vi "TimeSyncServ_Exec.vi"(8 "error in (no error)":errorcluster) -> ()   [LabVIEW 2019, in "PhotonVisionLib.lvlib"]
doc: "Execute a PhotonVision Time Sync Server. It listens for UDP requests from PhotonVision devices and responds with the current FPGA time.\n\nThis VI contains a loop. Do not place this in another loop.\n\nPlace this all by itself in Periodic Tasks.\n\n\nInputs:\n -- Error In -- Optional error input cluster.\n\nOutputs:\n -- <None>"
uses:
  PhotonVisionLib.lvlib
  <vilib>/Rock Robotics/WPI/ThirdParty/JAS_Junk/TrajLib/VI/Util_GetTime_U32.vi
  PhotonVision_Globals.vi
  <vilib>/Rock Robotics/WPI/ThirdParty/JAS_Junk/TrajLib/VI/Util_GetTime_U64.vi
  <vilib>/Rock Robotics/WPI/ThirdParty/JAS_Junk/TrajLib/Trajectory_Library.lvlib
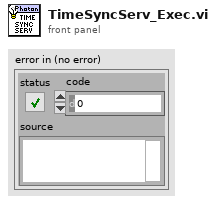
[diagram p1: front panel]
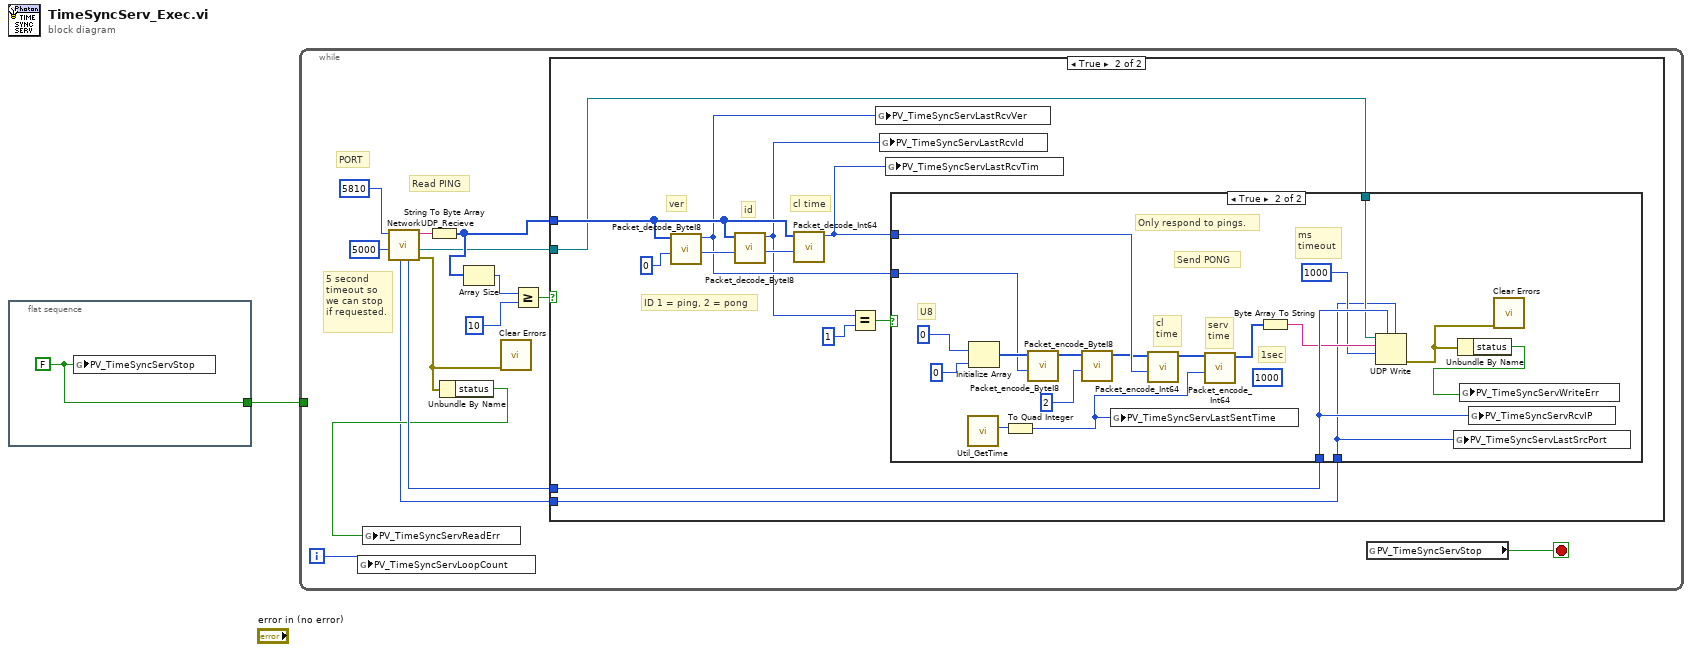
[diagram p0: block diagram]
diagram:
  n1 = flat-sequence {
    tunnel: [w2] -> w1
    frame #0 {
      w2 = FALSE ("PV_TimeSyncStopServ")
      n2 = global write "PhotonVision_Globals.vi" "PV_TimeSyncServStop"(w2) -> ()
    }
  }
  n3 = while {
    tunnel: w1 -> [_]
    i -> [w7]
    stop <- w8 stop-if-true
    # "Read PING"
    # "PORT"
    # "5 second\ntimeout so\nwe can stop\nif requested."
    n4 = global write "PhotonVision_Globals.vi" "PV_TimeSyncServLoopCount"(w7) -> ()
    n5 = call <vilib>:"NetworkUDP_Recieve.vi"("timeout ms (25000)"=5000, "receiver port"=u16 5810) -> ("error out"=w6:errorcluster, "UDP Network Connection out"=w3:refnum<k16>, "data out"=w14:string, "SenderAddress"=w10:u32, "SenderSrcPort"=w4:u16)  [unwired: 4 in, 1 out]
    n6 = String To Byte Array(string=w14) -> (unsigned byte array=w13:u8[])
    n7 = Unbundle By Name(w6) -> ("status"=w5:bool)
    n8 = global write "PhotonVision_Globals.vi" "PV_TimeSyncServReadErr"(w5) -> ()
    n9 = Array Size(array=w13) -> (size(s)=w12:i32)
    n10 = call <vilib>:"Clear Errors.vi"("error in (no error)"=w6) -> ()  [unwired: 5 in, 2 out]
    n11 = Greater Or Equal?(x=w12, y=10) -> (x >= y?=w15:bool)
    n12 = case shown="True" w15 {
      tunnel: w13 -> [_ w26]
      tunnel: w10 -> [_ w25]
      tunnel: w4 -> [_ w18]
      tunnel: w3 -> [_ w17]
      frame False {
      }
      frame True {
        # "ID 1 = ping, 2 = pong"
        # "cl time"
        # "id"
        # "ver"
        n13 = call "Packet_decode_ByteI8.vi"("StartByte"=0, "RawData"=w26) -> ("NextByte"=w27:i32, "Int8_Value"=w22:i8)  [unwired: 8 in]
        n14 = call "Packet_decode_ByteI8.vi"("StartByte"=w27, "RawData"=w26) -> ("NextByte"=w24:i32, "Int8_Value"=w20:i8)  [unwired: 8 in]
        n15 = call "Packet_decode_Int64.vi"("StartByte"=w24, "RawData"=w26) -> ("Int64_Value"=w23:i64)  [unwired: 8 in, 1 out]
        n16 = Equal?(x=w20, y=i8 1) -> (x = y?=w21:bool)
        n17 = global write "PhotonVision_Globals.vi" "PV_TimeSyncServLastRcvVer"(w22) -> ()
        n18 = global write "PhotonVision_Globals.vi" "PV_TimeSyncServLastRcvId"(w20) -> ()
        n19 = global write "PhotonVision_Globals.vi" "PV_TimeSyncServLastRcvTim"(w23) -> ()
        n20 = case shown="True" w21 {
          tunnel: w25 -> [_ w34]
          tunnel: w23 -> [_ w41]
          tunnel: w22 -> [_ w38]
          tunnel: w18 -> [_ w29]
          tunnel: w17 -> [_ w33]
          frame False {
          }
          frame True {
            (unwired) 1000 ("timeout ms (25000)")
            # "ms\ntimeout"
            # "1sec"
            # "Send PONG"
            # "Only respond to pings."
            # "serv\ntime"
            # "cl\ntime"
            # "U8"
            n21 = call <vilib>:"Util_GetTime.vi"() -> ("FPGA_Time_MicroSeconds"=w36:u64)  [unwired: 9 in, 2 out]
            n22 = Initialize Array(u8 0 ("element"), 0 ("dimension size")) -> (w43:u8[])
            n23 = To Quad Integer(1:w36) -> (0:w35:i64)
            n24 = call "Packet_encode_ByteI8.vi"("Int8_Value"=w38, "RawData In"=w43) -> ("RawData Out"=w47:u8[])  [unwired: 9 in]
            n25 = call "Packet_encode_ByteI8.vi"("Int8_Value"=i8 2, "RawData In"=w47) -> ("RawData Out"=w40:u8[])  [unwired: 9 in]
            n26 = global write "PhotonVision_Globals.vi" "PV_TimeSyncServLastSentTime"(w35) -> ()
            n27 = call "Packet_encode_Int64.vi"("Int64_Value"=w41, "RawData In"=w40) -> ("RawData Out"=w39:u8[])  [unwired: 9 in]
            n28 = call "Packet_encode_Int64.vi"("Int64_Value"=w35, "RawData In"=w39) -> ("RawData Out"=w46:u8[])  [unwired: 9 in]
            n29 = Byte Array To String(unsigned byte array=w46) -> (string=w32:string)
            n30 = UDP Write(address=w34, port or service name=w29, connection ID=w33, data in=w32, 9:1000 ("timeout ms (25000)")) -> (error out=w30:errorcluster)  [unwired: 1 in, 1 out]
            n31 = global write "PhotonVision_Globals.vi" "PV_TimeSyncServLastSrcPort"(w29) -> ()
            n32 = Unbundle By Name(w30) -> ("status"=w37:bool)
            n33 = global write "PhotonVision_Globals.vi" "PV_TimeSyncServWriteErr"(w37) -> ()
            n34 = global write "PhotonVision_Globals.vi" "PV_TimeSyncServRcvIP"(w34) -> ()
            n35 = call <vilib>:"Clear Errors.vi"("error in (no error)"=w30) -> ()  [unwired: 5 in, 2 out]
          }
        }
      }
    }
    n36 = global read "PhotonVision_Globals.vi" "PV_TimeSyncServStop"() -> (w8:bool)
  }
